vi "Create OPCUA Server Auto.vi"(8 "Error In":errorcluster, 11 "XML config File Path":path=path "D:/work/Project support in lanzhou/OPCUA XML/xml/server config.xml") -> (0 "Error Out":errorcluster, 1 "Parse Errors":string, 2 "server endpoint URL":string, 3 "OPC UA server refnum out":refnum<k21>, 4 "trusted client certfications":path[](array[path]))   [LabVIEW 2014, in "OPCUA XML(dev).lvlib"]
doc: "This example loads test configuration data from an XML file, and checks to see if it is valid against a specific schema. Select whether you want to load the valid or invalid file and run the VI to see the results."
uses:
  OPCUA XML(dev).lvlib
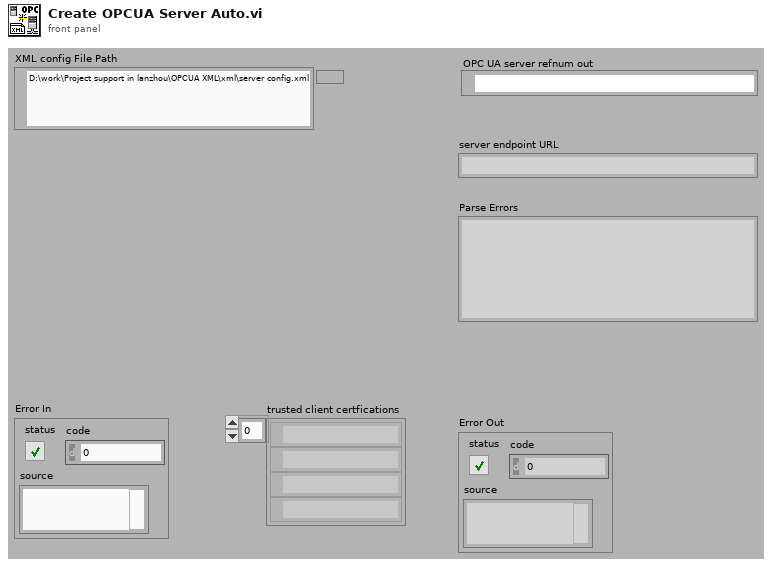
[diagram p1: front panel]
types:
  T1 = typedef "OPCUA XML(dev).lvlib/DEF-Server Config Data.ctl" = cluster{"name data":string, "port data":string, "policy data":string, "serverCertification data":string, "trustedClientCertifications data":string, "structure data":string}
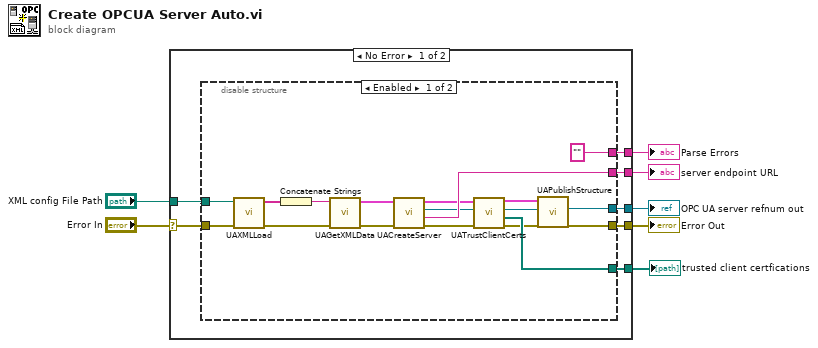
[diagram p0: block diagram]
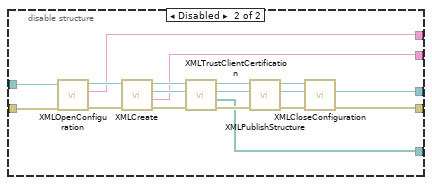
[diagram p2: hidden frame]
diagram:
  n1 = case shown="No Error" "Error In" {
    selector: "Error In" -> [w9 w51]
    tunnel: [w14 w51] -> w7
    tunnel: "XML config File Path" -> [w13 _]
    tunnel: [w12 _] -> w4
    tunnel: [w11 _] -> w3
    tunnel: [w10 _] -> w2
    tunnel: [w8 _] -> w1
    frame No Error {
      n2 = disable-structure shown="Enabled" {
        disable-tunnel: [w32 w38] -> w14
        disable-tunnel: w13 -> [w31 w34]
        disable-tunnel: ["" ("Parse Errors") w35] -> w12
        disable-tunnel: [w29 w37] -> w11
        disable-tunnel: [w28 w36] -> w10
        disable-tunnel: w9 -> [w27 w33]
        disable-tunnel: [w26 w39] -> w8
        frame Enabled {
          n3 = call "UAXMLLoad.vi"("error in (no error)"=w27, "XML File Path"=w31) -> ("error out"=w24:errorcluster, "xml Data"=w15:string[])  [unwired: 8 in]
          n4 = Concatenate Strings(w15) -> (w25:string)
          n5 = call "UAGetXMLData.vi"("error in (no error)"=w24, "String"=w25) -> ("error out"=w22:errorcluster, "Server config info"=w23:T1)  [unwired: 8 in]
          n6 = call "UACreateServer.vi"("error in (no error)"=w22, "Server config info"=w23) -> ("error out"=w21:errorcluster, "server endpoint URL"=w28:string, "OPC UA server refnum out"=w19:refnum<k21>, "Server config info (dup)"=w20:T1)  [unwired: 6 in]
          n7 = call "UATrustClientCerts.vi"("error in (no error)"=w21, "OPC UA server refnum in"=w19, "Server config info"=w20) -> ("error out"=w16:errorcluster, "Array"=w26:path[], "OPC UA server refnum out"=w18:refnum<k21>, "Server config info (dup)"=w17:T1)  [unwired: 5 in]
          n8 = call "UAPublishStructure.vi"("error in (no error)"=w16, "OPC UA server refnum in"=w18, "Server config info"=w17) -> ("error out"=w32:errorcluster, "OPC UA server refnum out"=w29:refnum<k21>)  [unwired: 6 in, 1 out]
        }
        frame Disabled {
          n9 = call "XMLOpenConfiguration.vi"("Error In"=w33, "path to XML document"=w34) -> ("Error Out"=w50:errorcluster, "Parse Errors"=w35:string, "DOM document out"=w49:refnum<k20>)  [unwired: 7 in]
          n10 = call "XMLCreate.vi"("Error In"=w50, "DOM document in"=w49) -> ("Error Out"=w44:errorcluster, "server endpoint URL"=w36:string, "OPC UA server refnum out"=w48:refnum<k21>, "DOM document out"=w46:refnum<k20>)  [unwired: 6 in]
          n11 = call "XMLTrustClientCertification.vi"("Error In"=w44, "OPC UA server refnum in"=w48, "DOM document in"=w46) -> ("Error Out"=w43:errorcluster, "trusted client certfications"=w39:path[], "OPC UA server refnum out"=w47:refnum<k21>, "DOM document out"=w45:refnum<k20>)  [unwired: 5 in]
          n12 = call "XMLPublishStructure.vi"("Error In"=w43, "OPC UA server refnum in"=w47, "DOM document in"=w45) -> ("Error Out"=w41:errorcluster, "OPC UA server refnum out"=w42:refnum<k21>, "DOM document out"=w40:refnum<k20>)  [unwired: 6 in]
          n13 = call "XMLCloseConfiguration.vi"("error in (no error)"=w41, "OPC UA server refnum in"=w42, "DOM document in"=w40) -> ("error out"=w38:errorcluster, "OPC UA server refnum out"=w37:refnum<k21>)  [unwired: 7 in]
        }
      }
    }
    frame Error {
    }
  }
  "Error Out" <- w7
  "Parse Errors" <- w4
  "server endpoint URL" <- w2
  "OPC UA server refnum out" <- w3
  "trusted client certfications" <- w1
